vi "RemoteVI Post Client Input.vi"(0 "panel":T3, 1 "kind":T2(ring), 2 "msg":u32, 3 "x":i32, 4 "y":i32, 5 "error in":errorcluster, 6 "wParam":u64, 7 "mods set":u8, 8 "lParam":i64, 9 "popup since":u32, 10 "popups":T1, 12 "mods":u8) -> (14 "tracking out":bool, 15 "clicked?":bool, 16 "popups out":T1, 17 "mods out":u8, 18 "mods set out":u8, 19 "error out":errorcluster)   [LabVIEW 2020, in "RemoteVI.lvlib"]
doc: "Posts one mouse or key message of a client to LabVIEW (docs\\protocol.md sections 4-6): a minimized panel is restored first (RemoteVI Restore If Minimized.vi); mods are updated (RemoteVI Track Modifiers.vi) and, when they changed and no popup is open, written into the key state of LabVIEW's UI thread (RemoteVI Apply Modifiers.vi); a WM_MOUSEMOVE while a popup is open is remembered for the menu hover (RemoteVI Note Popup Pointer.vi - RemoteVI Menu Hover.vi applies it once per server loop iteration); the message is translated (RemoteVI Translate Input.vi with the panel geometry, popup and tracking in = LabVIEW holds the mouse capture, RemoteVI Mouse Captured.vi) and posted to hWnd (RemoteVI Post Input.vi, which turns a click on a LabVIEW menu into keys and clicks other popups with the mouse path - popup since lets a mouse-path click wait until the popup is 350 ms old). Nothing here waits for the popup any more, so a click on a menu does not hold the server loop. clicked? is TRUE for anything but WM_MOUSEMOVE and WM_MOUSEWHEEL - a message that may open a popup. No VI Server call."
uses:
  RemoteVI.lvlib
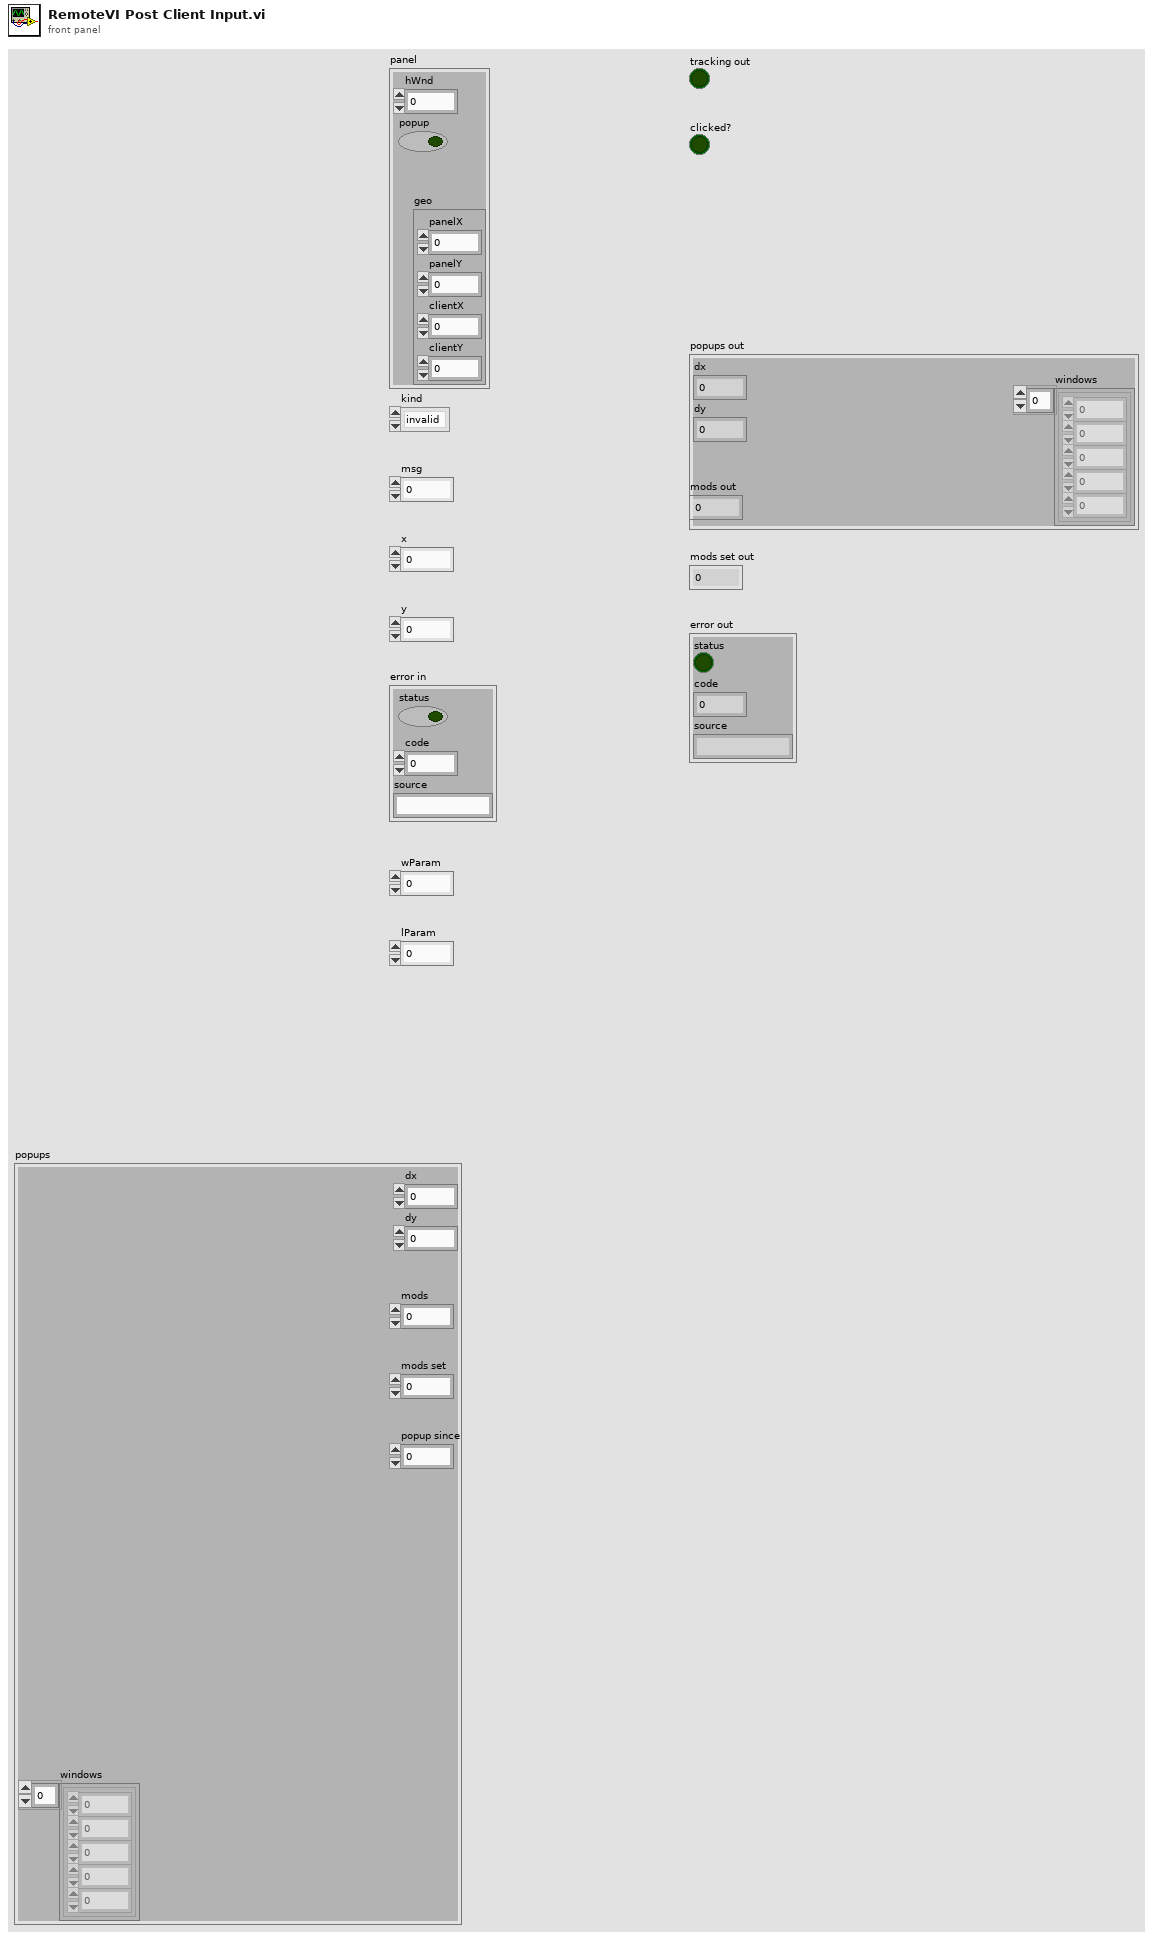
[diagram p1: front panel]
types:
  T1 = cluster{"windows":cluster{"hwnd":u64, "x":i32, "y":i32, "w":i32, "h":i32}[], "dx":i32, "dy":i32}
  T2 = enum16{"invalid", "mouse", "key", "ack", "close", "splitter"}
  T3 = cluster{"hWnd":u64, "popup":bool, "geo":cluster{"panelX":i32, "panelY":i32, "clientX":i32, "clientY":i32}}
  T4 = cluster{"panelX":i32, "panelY":i32, "clientX":i32, "clientY":i32}
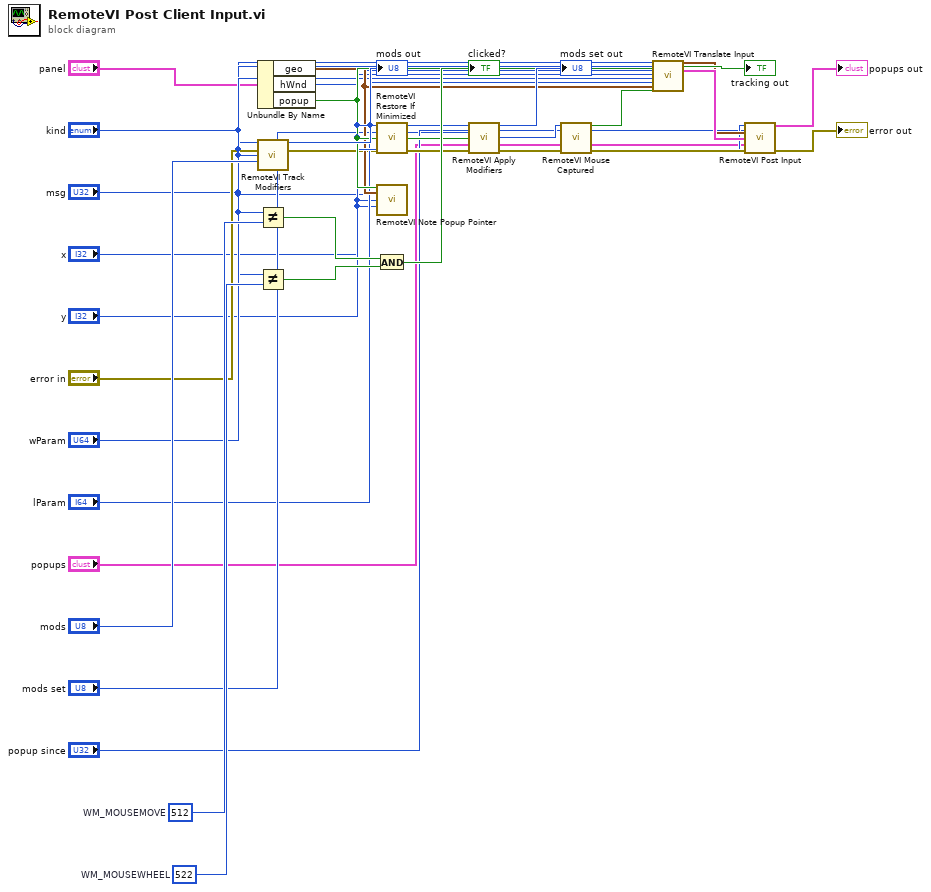
[diagram p0: block diagram]
diagram:
  w28 = u32 522  # WM_MOUSEWHEEL
  w27 = u32 512  # WM_MOUSEMOVE
  n1 = Unbundle By Name("panel") -> ("geo"=w13:T4, "hWnd"=w14:u64, "popup"=w15:bool)
  n2 = call "RemoteVI Track Modifiers.vi"("kind"="kind", "msg"="msg", "wParam"="wParam", "mods in"="mods") -> ("mods out"=w17:u8)  [unwired: 11 in]
  "mods out" <- w17
  n3 = Not Equal?(x="msg", y=w27) -> (x != y?=w29:bool)
  n4 = Not Equal?(x="msg", y=w28) -> (x != y?=w30:bool)
  n5 = call "RemoteVI Restore If Minimized.vi"("hWnd"=w14, "error in"="error in") -> ("error out"=w16:errorcluster)  [unwired: 12 in, 1 out]
  n6 = call "RemoteVI Note Popup Pointer.vi"("popup?"=w15, "geo"=w13, "msg"="msg", "x"="x", "y"="y") -> ()  [unwired: 11 in]
  n7 = And(x=w29, y=w30) -> (x .and. y?=→"clicked?":bool)
  n8 = call "RemoteVI Apply Modifiers.vi"("mods"=w17, "mods set"="mods set", "popup"=w15, "hWnd"=w14, "error in"=w16) -> ("mods set out"=→"mods set out":u8, "error out"=w19:errorcluster)  [unwired: 9 in]
  n9 = call "RemoteVI Mouse Captured.vi"("hWnd"=w14, "error in"=w19) -> ("captured?"=w20:bool, "error out"=w21:errorcluster)  [unwired: 12 in]
  n10 = call "RemoteVI Translate Input.vi"("kind"="kind", "msg"="msg", "x"="x", "y"="y", "wParam"="wParam", "lParam"="lParam", "geo"=w13, "tracking in"=w20, "popup"=w15) -> ("posts"=w22:cluster{"msg":u32, "wParam":u64, "lParam":i64}[], "tracking out"=→"tracking out":bool, "cursor"=w24:cluster{"move?":bool, "x":i32, "y":i32})  [unwired: 16 in]
  n11 = call "RemoteVI Post Input.vi"("hWnd"=w14, "popup since"="popup since", "posts"=w22, "cursor"=w24, "popups"="popups", "error in"=w21) -> ("popups out"=→"popups out":T1, "error out"=→"error out":errorcluster)  [unwired: 8 in]
